vi "Add When VIs.vi"(8 "error in (no error)":errorcluster, 11 "Mock Class Generator In":refnum<class "Mock Class Generator.lvclass">) -> (0 "error out":errorcluster, 2 "When VIs":path[](array[path]), 3 "Mock Class Generator Out":refnum<class "Mock Class Generator.lvclass">)   [LabVIEW 2020, in "Mock Class Generator.lvclass"]
uses:
  Mock Class Generator.lvclass
  Mock Class Generator.lvclass/Mock Class Generator.ctl
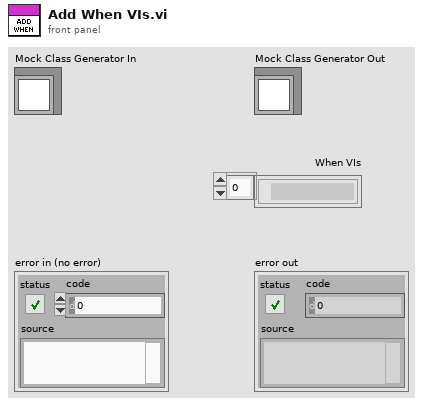
[diagram p1: front panel]
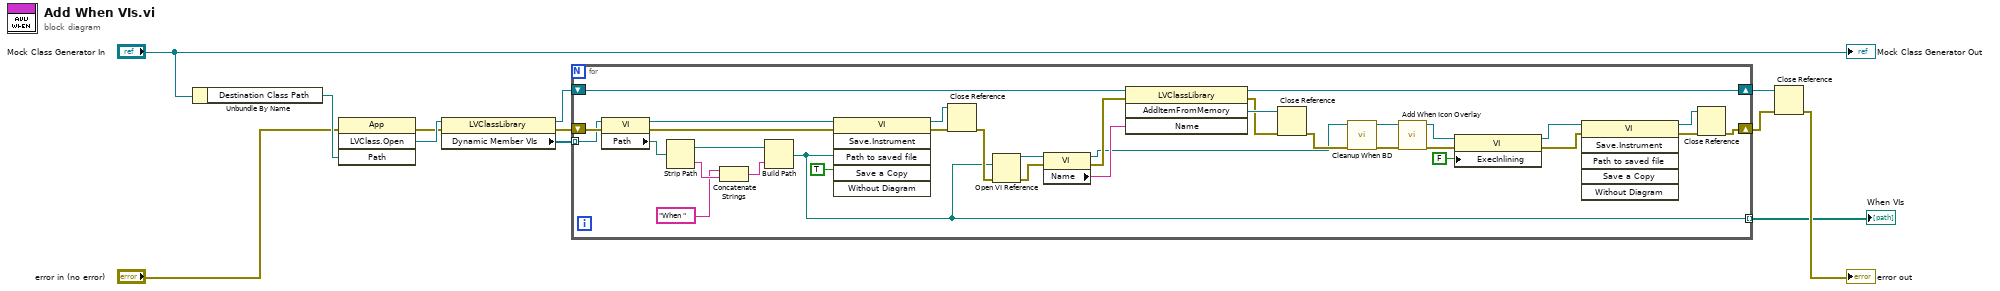
[diagram p0: block diagram]
diagram:
  n1 = Unbundle By Name("Mock Class Generator In") -> ("Destination Class Path"=w8:path)
  n2 = invoke class="App" method="LVClass.Open"(error in="error in (no error)", "Path"=w8) -> (error out=w11:errorcluster, "LVClass.Open"=w12:refnum<vi>)  [unwired: 2 in, 2 out]
  n3 = property class="LVClassLibrary"(reference=w12, error in=w11) -> (reference out=w6:refnum<vi>, error out=w10:errorcluster, "Dynamic Member VIs"=w7:refnum<vi>[])
  n4 = for {
    tunnel: w7 -> [w39] mode=indexing
    shift-right: [w21] -> w4
    shift-left: w10 -> [w40]
    shift-right: [w28] -> w5
    shift-left: w6 -> [w32]
    tunnel: [w20] -> w1 mode=indexing
    n5 = property class="VI"(reference=w39, error in=w40) -> (reference out=w44:refnum<vi>, error out=w43:errorcluster, "Path"=w46:path)
    n6 = Strip Path(path=w46) -> (stripped path=w38:path, name=w37:string)
    n7 = Concatenate Strings("When " ("string"), w37) -> (w35:string)
    n8 = Build Path(base path=w38, name or relative path=w35) -> (appended path=w20:path)
    n9 = invoke class="VI" method="Save.Instrument"(reference=w44, error in=w43, "Path to saved file"=w20, "Save a Copy"=TRUE) -> (reference out=w41:refnum<vi>, error out=w42:errorcluster)  [unwired: 2 in, 4 out]
    n10 = Close Reference(reference=w41, error in (no error)=w42) -> (error out=w31:errorcluster)
    n11 = Open VI Reference(vi path=w20, error in (no error)=w31) -> (vi reference=w30:refnum<vi>, error out=w29:errorcluster)  [unwired: 4 in]
    n12 = property class="VI"(reference=w30, error in=w29) -> (reference out=w22:refnum<vi>, error out=w33:errorcluster, "Name"=w34:string)
    n13 = invoke class="LVClassLibrary" method="AddItemFromMemory"(reference=w32, error in=w33, "Name"=w34) -> (reference out=w28:refnum<vi>, error out=w24:errorcluster, "AddItemFromMemory"=w25:refnum<vi>)  [unwired: 1 in, 1 out]
    n14 = Close Reference(reference=w25, error in (no error)=w24) -> (error out=w23:errorcluster)
    n15 = call "Cleanup When BD.vi"("error in (no error)"=w23, "VI in"=w22) -> ("error out"=w19:errorcluster, "VI out"=w18:refnum<vi>)  [unwired: 8 in]
    n16 = call "Add When Icon Overlay.vi"("error in (no error)"=w19, "VI in"=w18) -> ("error out"=w17:errorcluster, "VI out"=w15:refnum<vi>)  [unwired: 8 in]
    n17 = property class="VI"(reference=w15, error in=w17, "ExecInlining"=FALSE ("Execution:Inline SubVI")) -> (reference out=w14:refnum<vi>, error out=w16:errorcluster)
    n18 = invoke class="VI" method="Save.Instrument"(reference=w14, error in=w16) -> (reference out=w27:refnum<vi>, error out=w26:errorcluster)  [unwired: 4 in, 4 out]
    n19 = Close Reference(reference=w27, error in (no error)=w26) -> (error out=w21:errorcluster)
  }
  "When VIs" <- w1
  n20 = Close Reference(reference=w5, error in (no error)=w4) -> (error out=→"error out":errorcluster)
  "Mock Class Generator Out" <- "Mock Class Generator In"
